vi "Measurement UI.vi"() -> ()   [LabVIEW 2022 SP3, in "Stepped Frequency Sweep_Class D Amplifier_UI.lvlib"]
uses:
  Stepped Frequency Sweep_Class D Amplifier_UI.lvlib
  shared/controls/sweep profile.ctl
  shared/controls/units - snr.ctl
  shared/controls/units - ratio.ctl
  shared/controls/digital output level units.ctl
  shared/ui/controls/view.ctl
  shared/controls/regulation target.ctl
  shared/controls/regulation target value units.ctl
  UI State.ctl
  <vilib>/Utility/miscctls.llb/LVBoundsTypeDef.ctl
  <vilib>/Utility/miscctls.llb/LVPoint32TypeDef.ctl
  <vilib>/Utility/miscctls.llb/LVPointTypeDef.ctl
  Y axis data selection.ctl
  shared/ui/UI Helpers.lvlib
  shared/audio popup ui/Audio Popup UI.lvlib
  shared/controls/audio controls.lvlib
panel:
  in  "view legend":T1
  out "plot point":string
  out "Sweep graph":cluster{"frequency (Hz)":dbl[], "THD+N":dbl[]}[](graph)
  out "Time domain graph":waveform(dbl)(graph)
  out "Frequency domain graph":T2(graph)
  in  "digital serial cfg file":string
  out "amplitude (Vrms)":dbl[](array[numeric])
  out "output power (W)":dbl[](array[numeric])
  out "SFDR (dBc)":dbl[](array[numeric])
  out "gain":dbl[](array[numeric])
  out "dynamic range (dB)":dbl[](array[numeric])
  out "THD":dbl[](array[numeric])
  out "THD+N":dbl[](array[numeric])
  out "SNR":dbl[](array[numeric])
  out "amplitude (dBFS)":dbl[](array[numeric])
  out "frequency (Hz)":dbl[](array[numeric])
  in  "Configuration tab":T3(tab)
  out "digital serial file name":string
  in  "configure digital serial":bool
  in  "master clock channel list":string caption="Master Clock Channel"
  in  "digital channel list":string caption="Digital Audio Channel"
  in  "output level":dbl=-1.0 caption="Output level" format="%#_3f"
  in  "output level units":T4
  in  "min settling cycles":u32 caption="Minimum settling cycles"
  in  "min settling time (s)":dbl=0.1 caption="Minimum settling time" format="%#_6ps"
  in  "sweep profile":T5=enum."Logarithmic" caption="Profile"
  in  "number of steps":u32=20000 caption="Number of steps"
  in  "sweep start frequency (Hz)":dbl=20.0 caption="Sweep start" format="%#_6pHz"
  in  "sweep stop frequency (Hz)":dbl=20000.0 caption="Sweep stop" format="%#_6pHz"
  in  "min measurement cycles":u32 caption="Minimum measurement cycles"
  in  "Acquisition channel":tag
  in  "acq sampling rate":dbl=51200.0 caption="Sample rate" format="%#.6pHz"
  in  "min measurement time (s)":dbl=0.1 caption="Minimum measurement time" format="%#_6ps"
  in  "lowpass filter":T6(ring) caption="Lowpass filter"
  in  "highpass filter":enum32{"DC", "AC"}(ring) caption="Highpass filter"
  in  "band start":dbl=20.0 caption="Band start" format="%#_6pHz"
  in  "band stop":dbl=20000.0 caption="Band stop" format="%#_6pHz"
  in  "weighting filter":T7(ring)=enum."A-weighting" caption="Weighting filter"
  in  "load impedance":dbl=4.0 caption="Load impedance" format="%#_6p Ohms"
  in  "output range (pk-pk)":dbl=15.0 caption="Output range" format="%.3p Vpk-pk"
  in  "regulation stop level":dbl=90.0 caption="Stop Level"
  in  "regulation output level units (stop)":T4
  in  "regulation target value units":T8 caption="Units"
  in  "regulation target value":dbl=20.0 caption="Target Value"
  in  "regulation target":T9 caption="Regulate"
  in  "enable regulation":bool caption="Enable Regulation"
  in  "regulation number of steps":u32=2 caption="Number of steps"
  in  "regulation start level":dbl=10.0 caption="Start Level"
  in  "regulation output level units":T4
  in  "gain units":T10 caption="Gain"
  in  "THD units":T10 caption="THD"
  in  "THD+N units":T10 caption="THD+N"
  in  "SNR units":T11 caption="SNR"
  in  "x-axis mapping":enum32{"linear", "logarithmic"}(ring) caption="X-axis mapping"
  in  "y-axis mapping":enum32{"linear", "logarithmic"}(ring) caption="Y-axis mapping"
  in  "channel 0 offset":u32=1
  out "fft - data":dbl[](array[numeric])
  out "fft - df":dbl
  out "fft - f0":dbl
  out "wfm - data":dbl[](array[numeric])
  out "wfm - dt":dbl
  out "wfm - t0":dbl
  out "channel name":string
  in  "acq channel":string="PXI1Slot4/ai0"
  in  "signal phase":dbl caption="phase"
  # "hidden controls - used to sync with MeasLink"
  # "hidden indicators"
  # "Digital Serial Settings"
  # "Harware Resource"
  # "Sweep"
  # "Filters"
  # "Output"
  # "Acquisition"
  # "Regulation"
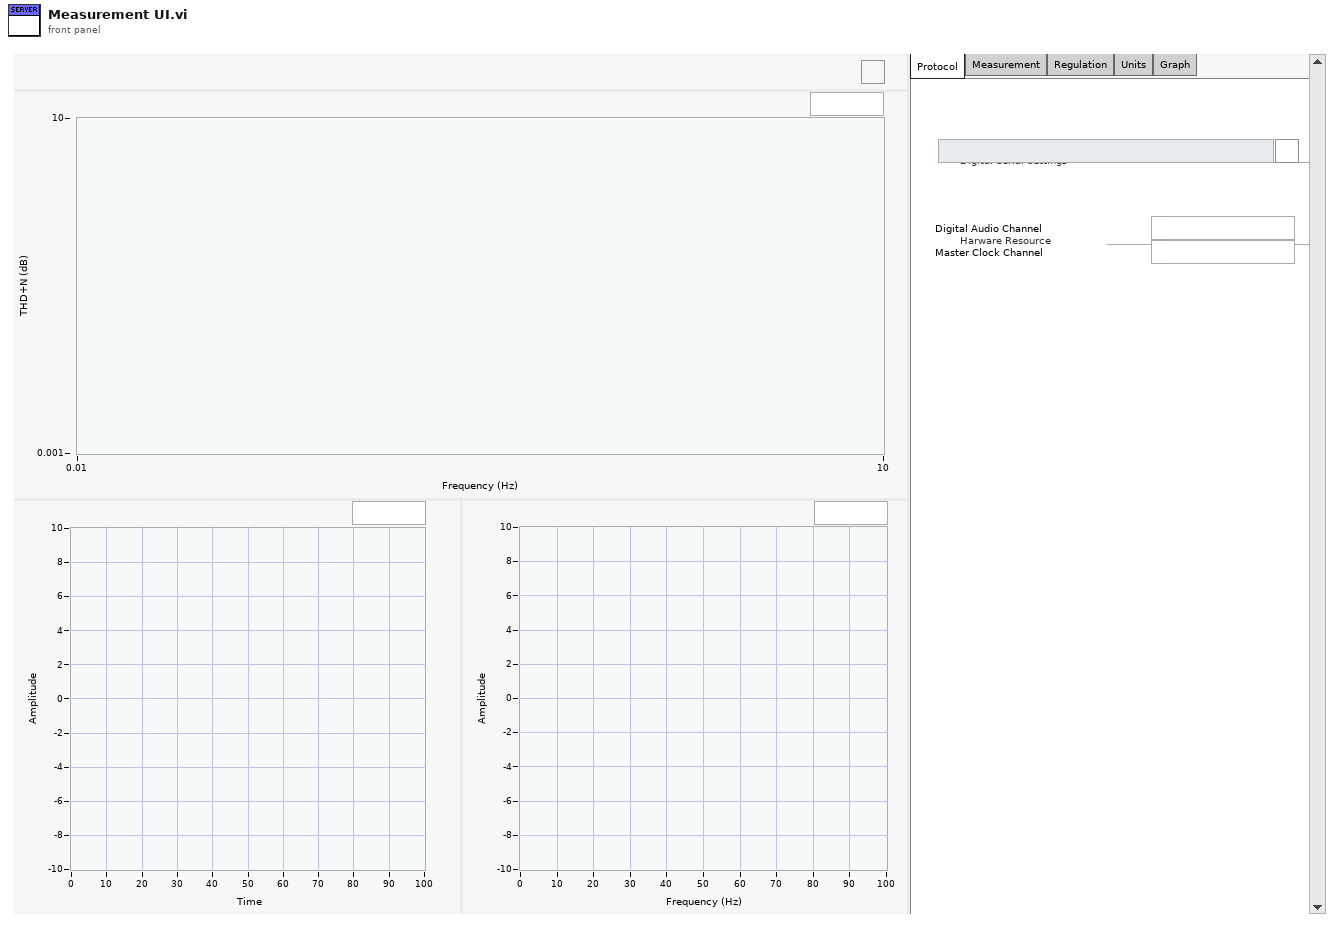
[diagram p1: front panel]
types:
  T1 = typedef "UI Helpers.lvlib/view.ctl" = bool
  T2 = cluster{"fft - f0":dbl, "fft - df":dbl, "fft - data":dbl[]}
  T3 = enum32{"Protocol", "Measurement", "Regulation", "Units", "Graph"}
  T4 = typedef "audio controls.lvlib/digital output level units.ctl" = enum32{"% FS", "dBFS", "V"}
  T5 = typedef "audio controls.lvlib/sweep profile.ctl" = enum32{"Linear", "Logarithmic"}
  T6 = enum32{"No filter", "AES17 20kHz", "AES17 40kHz"}
  T7 = enum32{"Linear", "A-weighting", "B-weighting", "C-weighting"}
  T8 = typedef "regulation target value units.ctl" = enum32{"%", "W"}
  T9 = typedef "regulation target.ctl" = enum32{"THD+N Ratio", "Output Power"}
  T10 = typedef "audio controls.lvlib/units - ratio.ctl" = enum32{"dB", "%", "x/y"}
  T11 = typedef "audio controls.lvlib/units - snr.ctl" = enum32{"dB", "x/y"}
  T12 = typedef "Stepped Frequency Sweep_Class D Amplifier_UI.lvlib/UI State.ctl" = cluster{"Graph Size":T13, "Legend Visible":bool, "Mouse Coords":T14, "Visible Plot Id":i32, "PostUI event occurred":bool, "digital serial cfg file":path}
  T13 = typedef "LVBoundsTypeDef.ctl" = cluster{"Width":u32, "Height":u32}
  T14 = typedef "LVPoint32TypeDef.ctl" = cluster{"Horizontal":i32, "Vertical":i32}
  T15 = typedef "LVPointTypeDef.ctl" = cluster{"Horizontal":i16, "Vertical":i16}
  T16 = typedef "Stepped Frequency Sweep_Class D Amplifier_UI.lvlib/Y axis data selection.ctl" = enum32{"THD+N", "THD", "SNR", "Gain", "Amplitude (dBFS)", "Amplitude (Vrms)", "Output Power (W)", "Dynamic Range (dB)", "SFDR (dBc)"}
  T17 = typedef "Audio Popup UI.lvlib/audio settings.ctl" = cluster{"digital serial file":string}
  T18 = cluster{"frequency (Hz)":dbl[], "amplitude (dBFS)":dbl[]}
  T19 = cluster{"frequency (Hz)":dbl[], "amplitude (Vrms)":dbl[]}
  T20 = cluster{"frequency (Hz)":dbl[], "output power (W)":dbl[]}
  T21 = cluster{"frequency (Hz)":dbl[], "dynamic range (dB)":dbl[]}
  T22 = cluster{"frequency (Hz)":dbl[], "SFDR (dBc)":dbl[]}
  T23 = cluster{"frequency (Hz)":dbl[], "SFDR (dBc)":dbl[]}[]
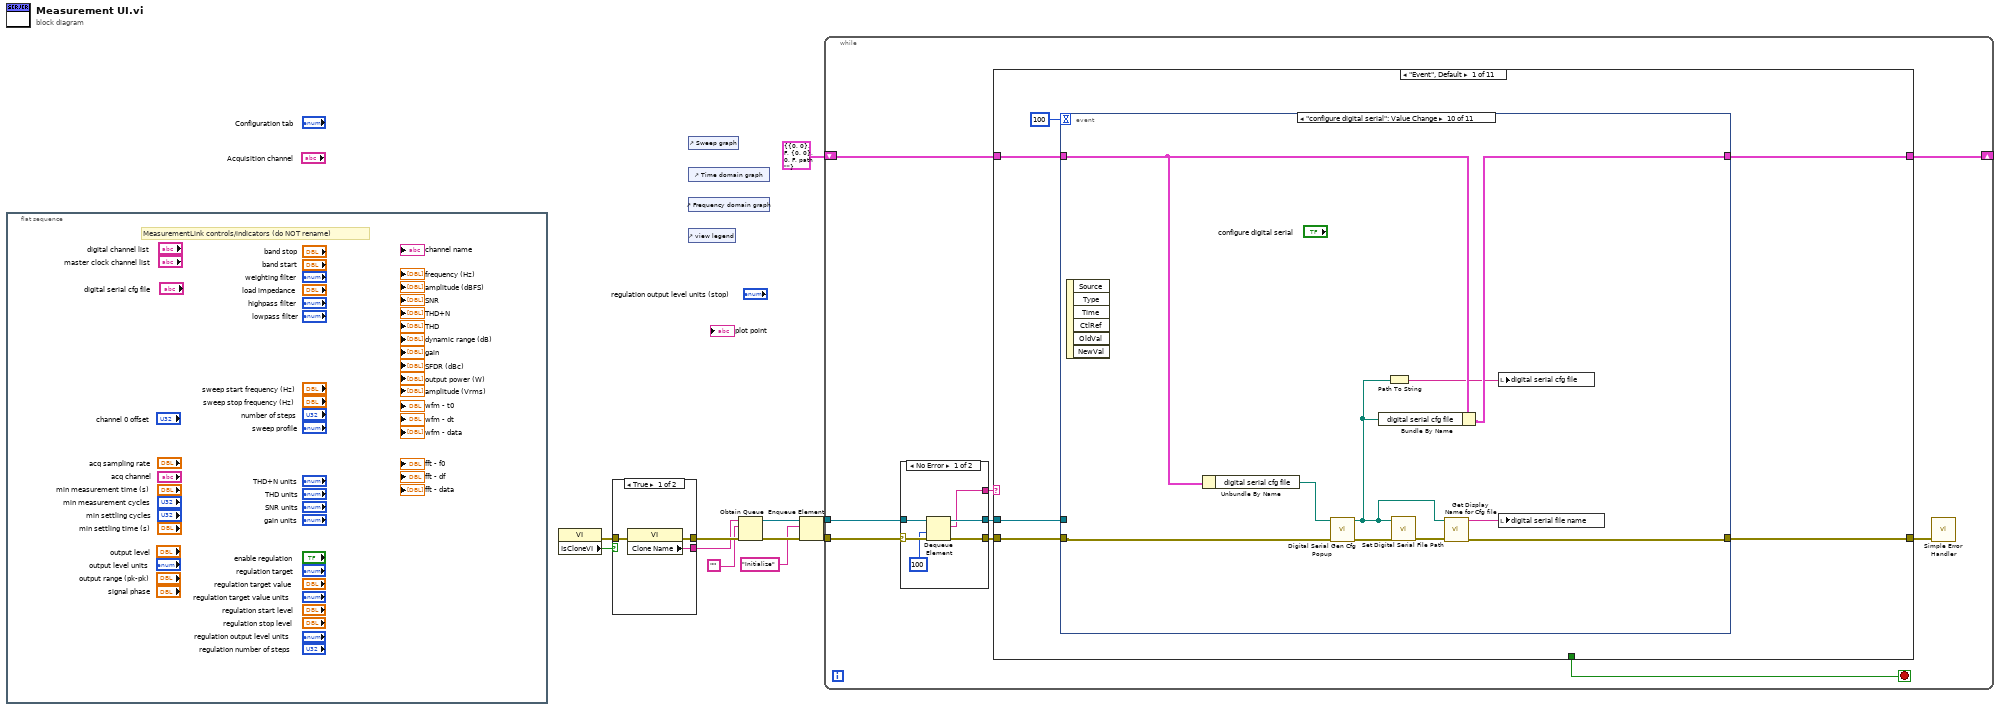
[diagram p0: block diagram]
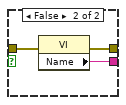
[diagram p2: hidden frame]
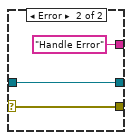
[diagram p3: hidden frame]
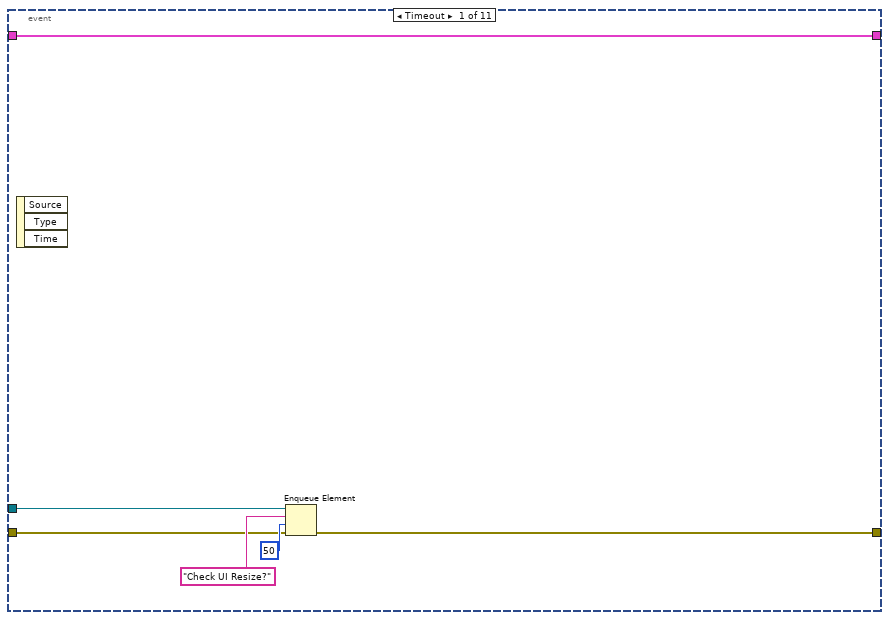
[diagram p4: hidden frame]
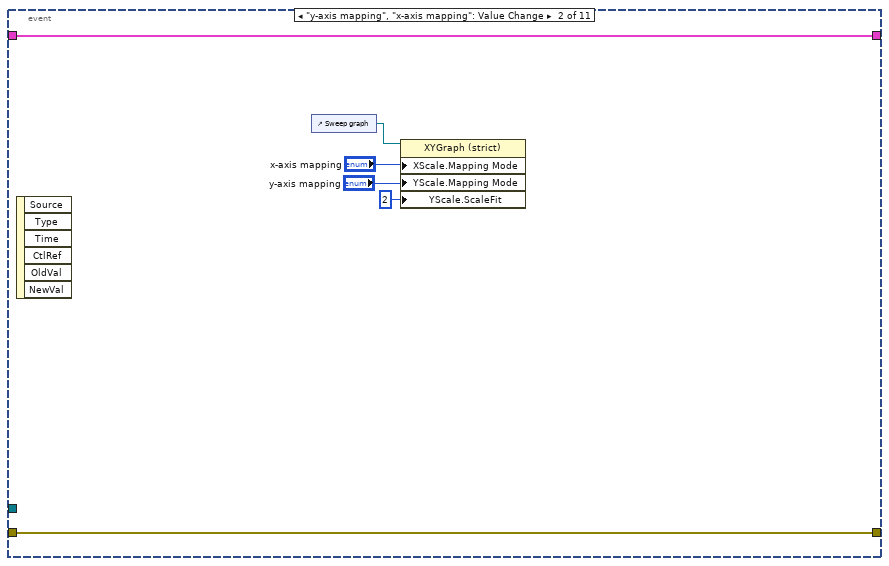
[diagram p5: hidden frame]
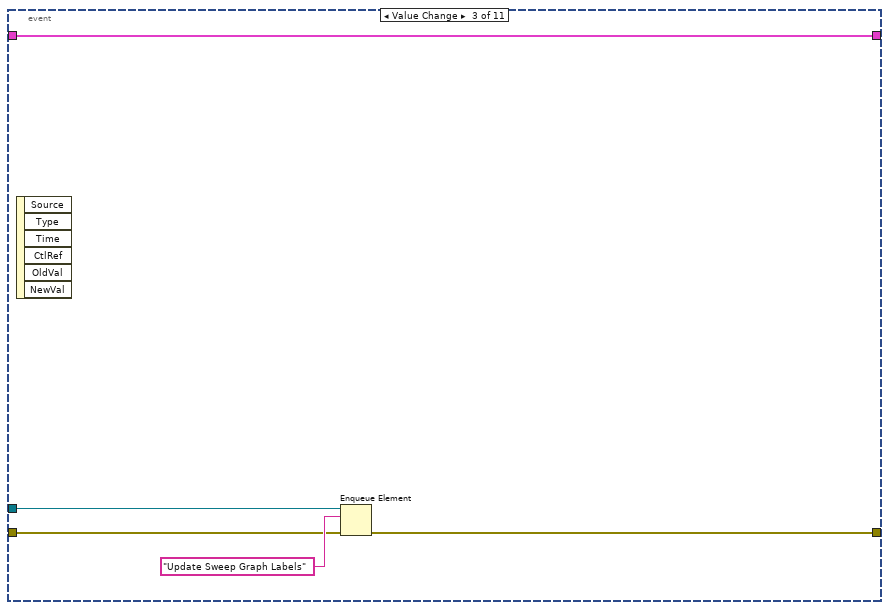
[diagram p6: hidden frame]
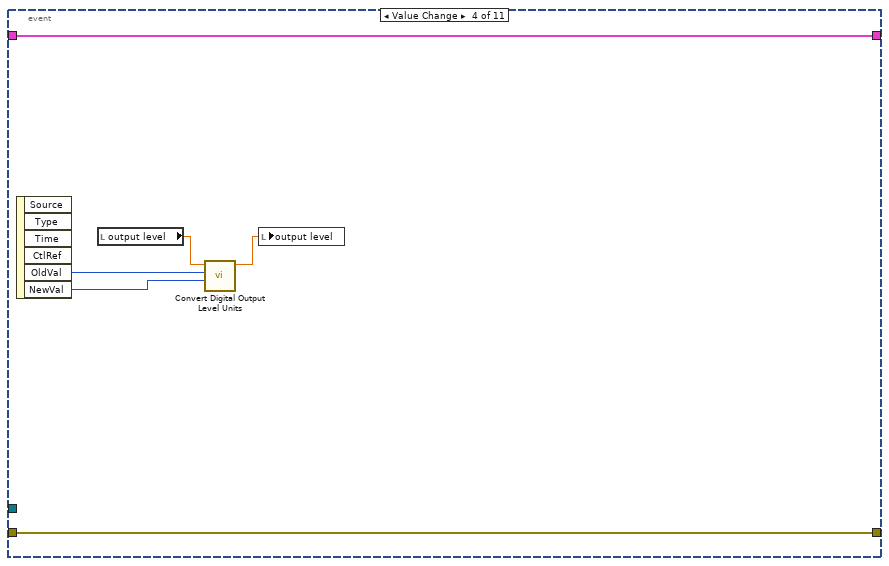
[diagram p7: hidden frame]
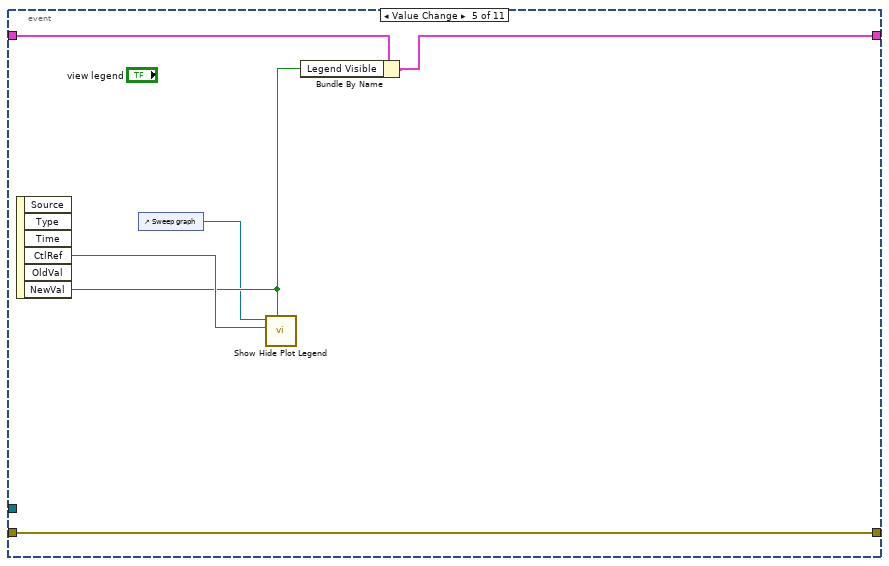
[diagram p8: hidden frame]
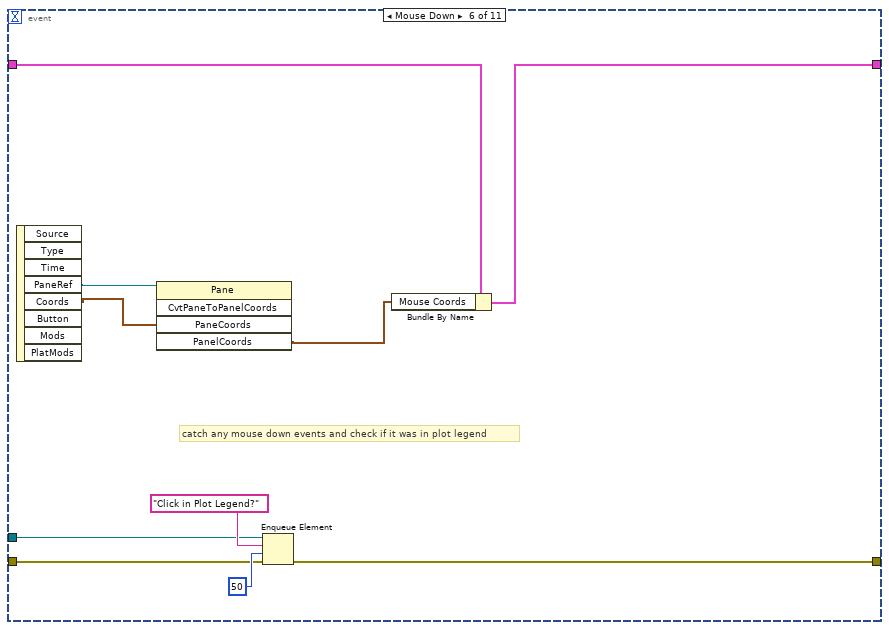
[diagram p9: hidden frame]
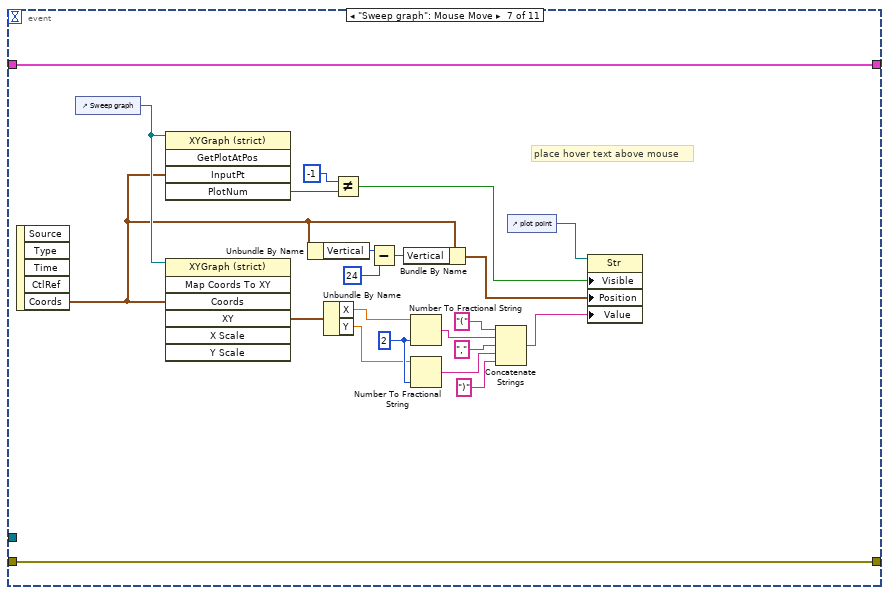
[diagram p10: hidden frame]
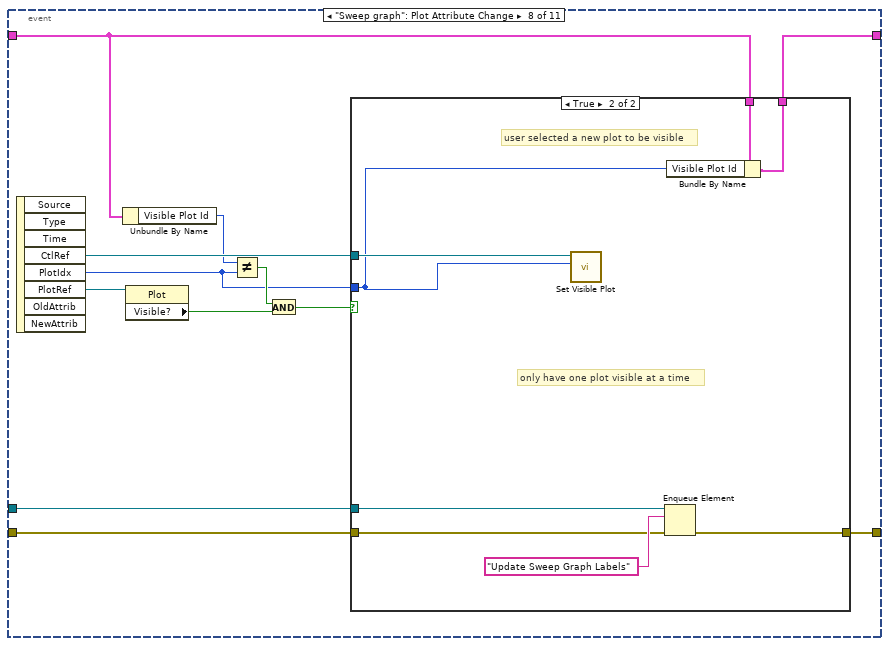
[diagram p11: hidden frame]
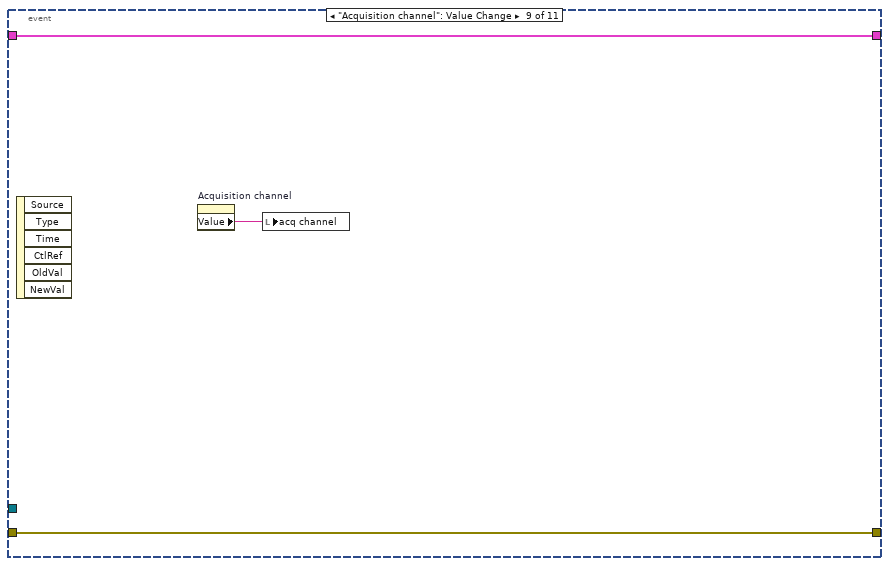
[diagram p13: hidden frame]
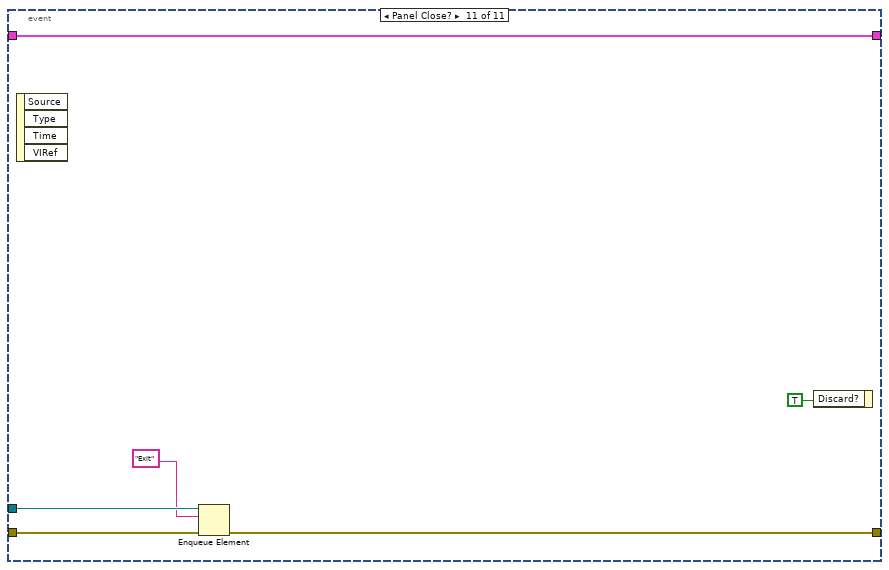
[diagram p14: hidden frame]
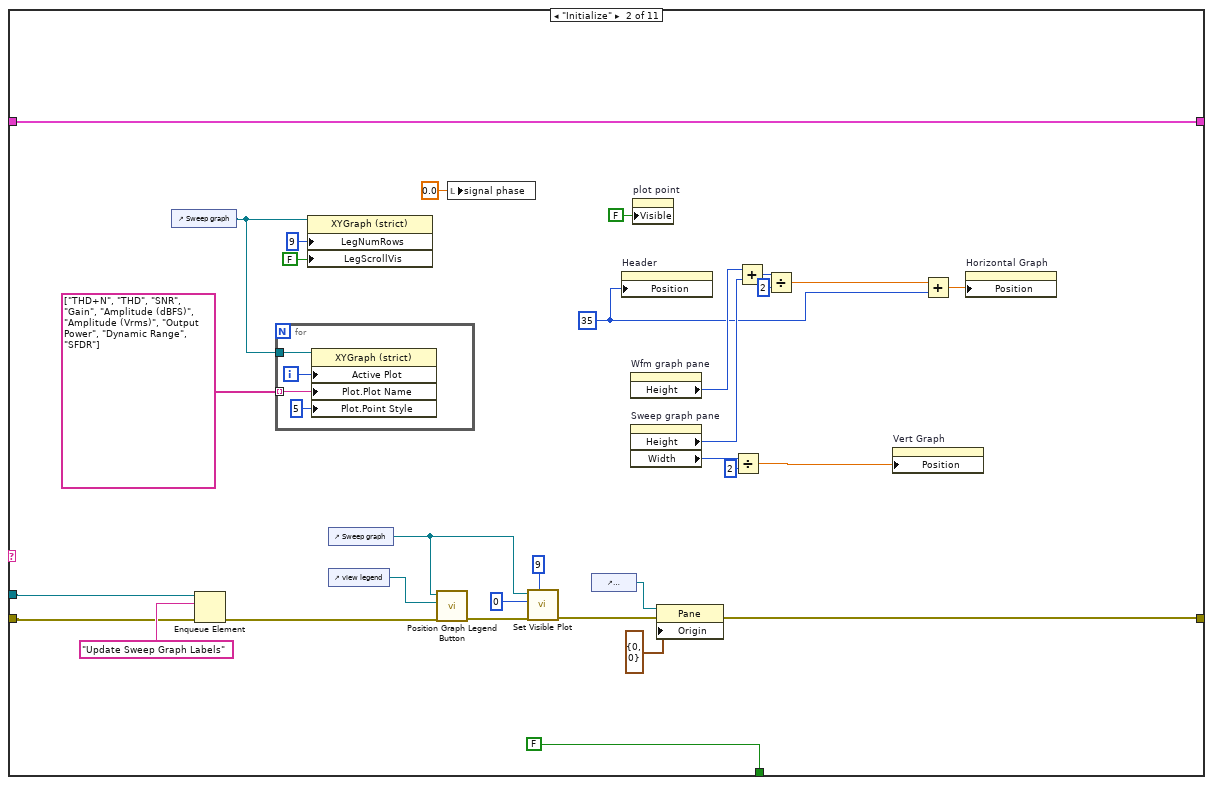
[diagram p15: hidden frame]
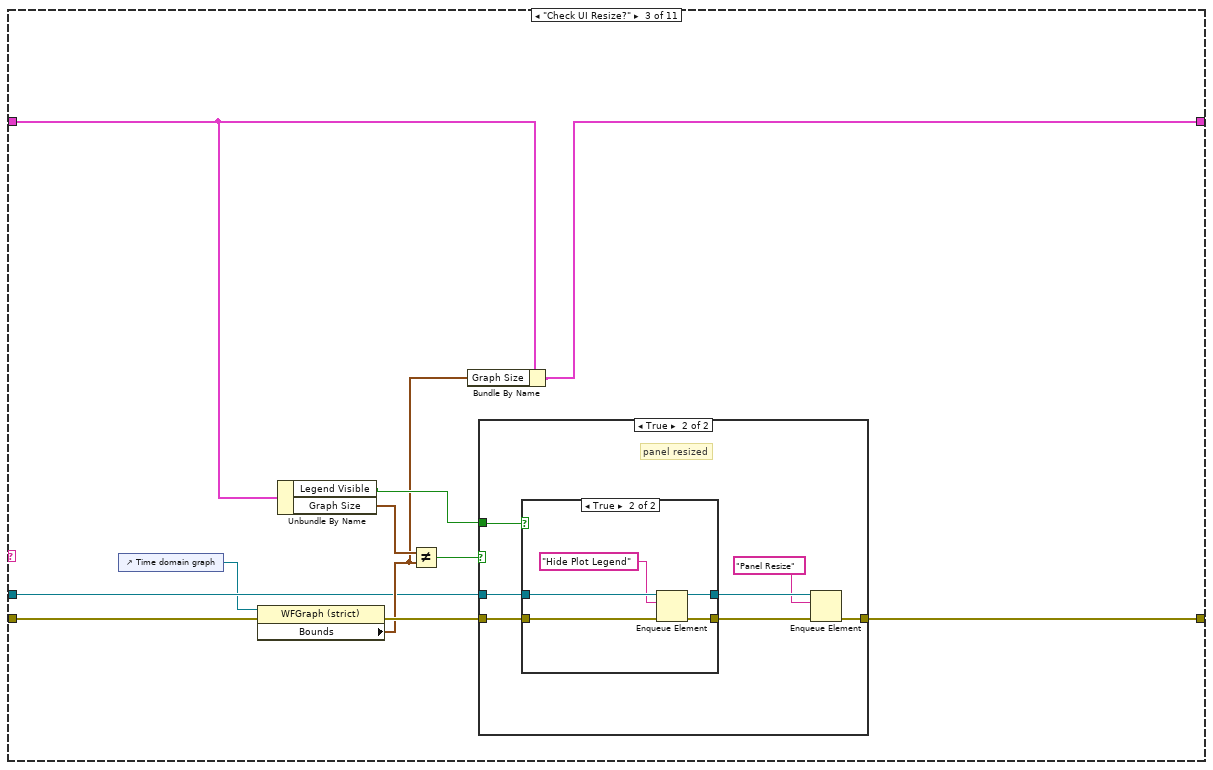
[diagram p16: hidden frame]
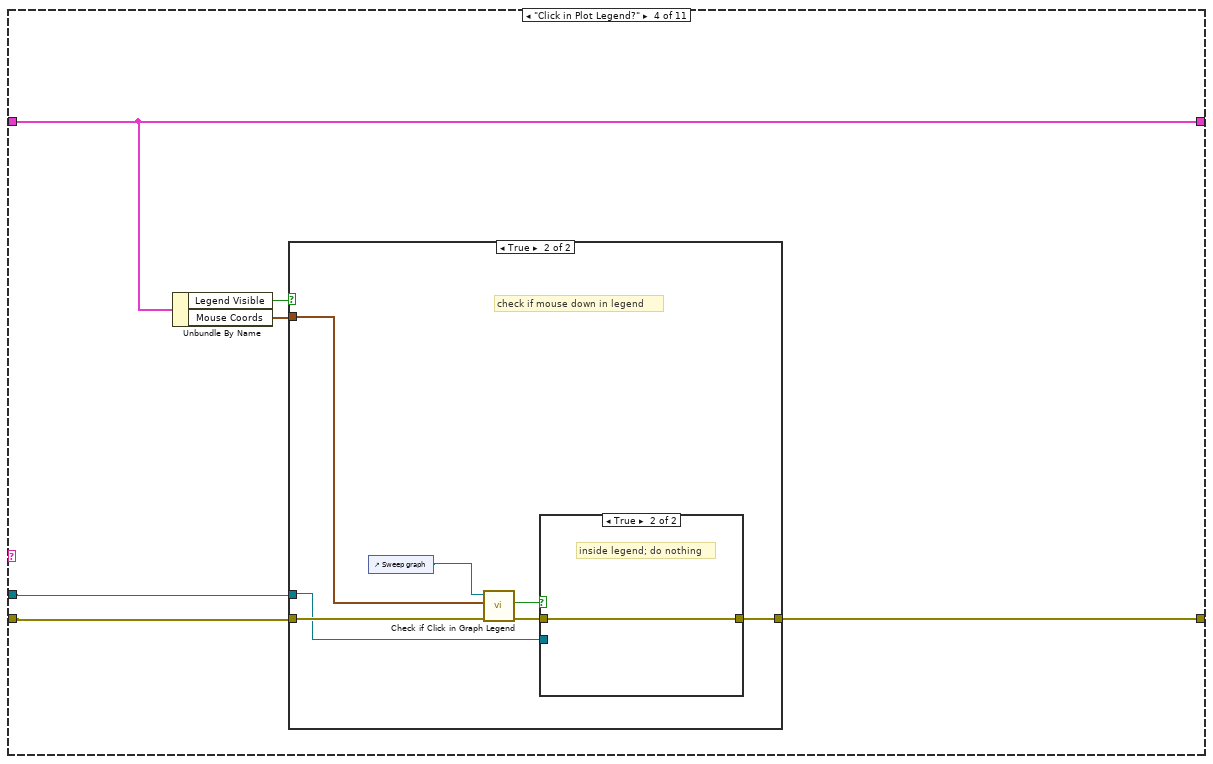
[diagram p19: hidden frame]
diagram:
  n1 = flat-sequence {
    frame #0 {
      # "MeasurementLink controls/indicators (do NOT rename)"
    }
  }
  n2 = property class="VI"() -> (error out=w2:errorcluster, "IsCloneVI"=w3:bool)  [unwired: 2 in, 1 out]
  n3 = case shown="True" w3 {
    tunnel: [w14 w17] -> w11
    tunnel: [w13 w16] -> w10
    tunnel: w2 -> [w12 w15]
    frame True {
      n4 = property class="VI"(error in=w12) -> (error out=w14:errorcluster, "Clone Name"=w13:string)  [unwired: 1 in, 1 out]
    }
    frame False {
      n5 = property class="VI"(error in=w15) -> (error out=w17:errorcluster, "Name"=w16:string)  [unwired: 1 in, 1 out]
    }
  }
  n6 = control-ref of="Sweep graph"() -> ()  [unwired: 1 out]
  n7 = control-ref of="Time domain graph"() -> ()  [unwired: 1 out]
  n8 = control-ref of="Frequency domain graph"() -> ()  [unwired: 1 out]
  n9 = control-ref of="view legend"() -> ()  [unwired: 1 out]
  n10 = Obtain Queue(name (unnamed)=w10, element data type="", error in (no error)=w11) -> (queue out=w7:refnum<queue>, error out=w9:errorcluster)  [unwired: 2 in, 1 out]
  n11 = Enqueue Element(queue=w7, element="Initialize", error in (no error)=w9) -> (queue out=w6:refnum<queue>, error out=w8:errorcluster)  [unwired: 1 in, 1 out]
  n12 = while {
    tunnel: w6 -> [w24]
    shift-right: [w20] -> _
    shift-left: T12 {"Graph Size"={"Width"=0, "Height"=0}, "Legend Visible"=FALSE, "Mouse Coords"={"Horizontal"=0, "Vertical"=0}, "Visible Plot Id"=0, "PostUI event occurred"=FALSE, "digital serial cfg file"=path ""} ("UI State") -> [w19]
    tunnel: w8 -> [w26]
    stop <- w21 stop-if-true
    n13 = case shown="No Error" w26 {
      selector: w26 -> [w32 w35]
      tunnel: [w31 w35] -> w25
      tunnel: w24 -> [w30 w34]
      tunnel: [w29 w34] -> w23
      tunnel: [w28 "Handle Error"] -> w22
      frame No Error {
        n14 = Dequeue Element(queue=w30, timeout in ms (-1)=100, error in (no error)=w32) -> (queue out=w29:refnum<queue>, element=w28:string, error out=w31:errorcluster)  [unwired: 1 out]
      }
      frame Error {
      }
    }
    n15 = case shown="\"Event\", Default" w22 {
      tunnel: w25 -> [w40 w152 w183 w207 w227 w235 w243 w291 w303 w316 w318]
      tunnel: w23 -> [w38 w153 w184 w208 _ _ w242 _ _ w314 _]
      tunnel: [w41 w148 w182 w206 w226 w234 w237 w291 w303 w311 w318] -> w18
      tunnel: [_ FALSE _ _ _ _ _ _ _ TRUE _] -> w21
      tunnel: [w36 w144 w179 w205 w229 w236 w240 w290 w302 w309 w317] -> w20
      tunnel: w19 -> [w37 w144 w180 w205 w230 w236 w241 w290 w302 w309 w317]
      frame "Event", Default {
        n16 = event shown="[9] \"configure digital serial\": Value Change" {
          selector: _ -> [_ _ _ _ _ _ _ _ _ _ _]
          dyn-events: _ -> [_ _ _ _ _ _ _ _ _ _ _]
          timeout: 100 -> [_ _ _ _ _ _ _ _ _ _ _]
          tunnel: [w44 w48 w54 w59 w70 w76 w102 w110 w125 w132 w141] -> w41
          tunnel: w40 -> [w45 w48 w55 w59 w70 w78 w102 w112 w125 w133 w142]
          tunnel: w38 -> [w43 _ w56 _ _ w77 _ w111 _ _ w140]
          tunnel: w37 -> [w42 w49 w58 w60 w67 w75 w101 w105 w126 w131 w138]
          tunnel: [w42 w49 w58 w60 w66 w74 w101 w104 w126 w130 w138] -> w36
          event Timeout {
            n17 = event-data() -> ()  [unwired: 1 in, 3 out]
            n18 = Enqueue Element(queue=w43, element="Check UI Resize?", timeout in ms (-1)=50, error in (no error)=w45) -> (error out=w44:errorcluster)  [unwired: 2 out]
          }
          event "y-axis mapping", "x-axis mapping": Value Change {
            n19 = event-data() -> ()  [unwired: 1 in, 6 out]
            n20 = control-ref of="Sweep graph"() -> (w51:refnum<vi>)
            n21 = property on="Property Node" class="XYGraph (strict)"(reference=w51, "XScale.Mapping Mode"="x-axis mapping", "YScale.Mapping Mode"="y-axis mapping", "YScale.ScaleFit"=u8 2 ("Y Scale.Scale Fit")) -> ()  [unwired: 1 in, 2 out]
          }
          event Value Change {
            n22 = event-data() -> ()  [unwired: 1 in, 6 out]
            n23 = Enqueue Element(queue=w56, element="Update Sweep Graph Labels", error in (no error)=w55) -> (error out=w54:errorcluster)  [unwired: 1 in, 2 out]
          }
          event Value Change {
            n24 = event-data() -> ("OldVal"=w64:T4, "NewVal"=w63:T4)  [unwired: 1 in, 4 out]
            n25 = local read "output level"() -> (w61:dbl)
            n26 = call "Convert Digital Output Level Units.vi"("new output level units"=w63, "previous output level units"=w64, "previous output level"=w61) -> ("new output level"=w62:dbl)  [unwired: 8 in]
            n27 = local write "output level"(w62) -> ()
          }
          event Value Change {
            n28 = event-data() -> ("CtlRef"=w69:refnum<vi>, "NewVal"=w68:T1)  [unwired: 1 in, 4 out]
            n29 = control-ref of="Sweep graph"() -> (w65:refnum<vi>)
            n30 = call "Show Hide Plot Legend.vi"("show"=w68, "view reference"=w69, "graph reference"=w65) -> ()  [unwired: 8 in, 1 out]
            n31 = Bundle By Name(cluster=w67, "Legend Visible"=w68) -> (w66:T12)
          }
          event Mouse Down {
            # "catch any mouse down events and check if it was in plot legend"
            n32 = event-data() -> ("PaneRef"=w73:refnum<vi>, "Coords"=w72:T14)  [unwired: 1 in, 6 out]
            n33 = invoke class="Pane" method="CvtPaneToPanelCoords"(reference=w73, "PaneCoords"=w72) -> ("PanelCoords"=w71:T15)  [unwired: 3 in, 4 out]
            n34 = Enqueue Element(queue=w77, element="Click in Plot Legend?", timeout in ms (-1)=50, error in (no error)=w78) -> (error out=w76:errorcluster)  [unwired: 2 out]
            n35 = Bundle By Name(cluster=w75, "Mouse Coords"=w71) -> (w74:T12)
          }
          event "Sweep graph": Mouse Move {
            w91 = i16 2 ("precision (6)")
            # "place hover text above mouse"
            n36 = event-data() -> ("Coords"=w86:T14)  [unwired: 1 in, 4 out]
            n37 = control-ref of="Sweep graph"() -> (w87:refnum<vi>)
            n38 = invoke class="XYGraph (strict)" method="GetPlotAtPos"(reference=w87, "InputPt"=w86) -> ("PlotNum"=w99:i32)  [unwired: 3 in, 4 out]
            n39 = invoke class="XYGraph (strict)" method="Map Coords To XY"(reference=w87, "Coords"=w86) -> ("XY"=w100:cluster{"X":dbl, "Y":dbl})  [unwired: 5 in, 6 out]
            n40 = Unbundle By Name(w86) -> ("Vertical"=w84:i32)
            n41 = Unbundle By Name(w100) -> ("X"=w89:dbl, "Y"=w88:dbl)
            n42 = Not Equal?(x=-1, y=w99) -> (x != y?=w97:bool)
            n43 = Subtract(x=w84, y=24) -> (x-y=w83:i32)
            n44 = Bundle By Name(cluster=w86, "Vertical"=w83) -> (w85:T14)
            n45 = Number To Fractional String(number=w89, precision (6)=w91) -> (F-format string=w95:string)  [unwired: 2 in]
            n46 = Number To Fractional String(number=w88, precision (6)=w91) -> (F-format string=w93:string)  [unwired: 2 in]
            n47 = Concatenate Strings("(" ("string"), w95, "," ("string"), w93, ")" ("string")) -> (w90:string)
            n48 = control-ref of="plot point"() -> (w81:refnum<vi>)
            n49 = property on="Property Node" class="Str"(reference=w81, "Visible"=w97, "Position"=w85, "Value"=w90) -> ()  [unwired: 1 in, 2 out]
          }
          event "Sweep graph": Plot Attribute Change {
            n50 = event-data() -> ("CtlRef"=w113:refnum<vi>, "PlotIdx"=w103:i32, "PlotRef"=w114:refnum<vi>)  [unwired: 1 in, 5 out]
            n51 = Unbundle By Name(w105) -> ("Visible Plot Id"=w109:i32)
            n52 = property class="Plot"(reference=w114) -> ("Visible?"=w107:bool)  [unwired: 1 in, 2 out]
            n53 = Not Equal?(x=w109, y=w103) -> (x != y?=w108:bool)
            n54 = And(x=w108, y=w107) -> (x .and. y?=w106:bool)
            n55 = case shown="True" w106 {
              tunnel: w113 -> [_ w124]
              tunnel: w112 -> [w116 w122]
              tunnel: w111 -> [_ w121]
              tunnel: [w116 w120] -> w110
              tunnel: w105 -> [w115 w119]
              tunnel: [w115 w118] -> w104
              tunnel: w103 -> [_ w117]
              frame False {
              }
              frame True {
                # "only have one plot visible at a time"
                # "user selected a new plot to be visible"
                n56 = call "Set Visible Plot.vi"("Plot Id"=w117, "XYGraph in"=w124) -> ()  [unwired: 9 in, 1 out]
                n57 = Enqueue Element(queue=w121, element="Update Sweep Graph Labels", error in (no error)=w122) -> (error out=w120:errorcluster)  [unwired: 1 in, 2 out]
                n58 = Bundle By Name(cluster=w119, "Visible Plot Id"=w117) -> (w118:T12)
              }
            }
          }
          event "Acquisition channel": Value Change {
            n59 = event-data() -> ()  [unwired: 1 in, 6 out]
            n60 = property on="Acquisition channel" class="DAQmxName"() -> ("Value"=w127:string)  [unwired: 2 in, 2 out]
            n61 = local write "acq channel"(w127) -> ()
          }
          event "configure digital serial": Value Change {
            n62 = event-data() -> ()  [unwired: 1 in, 6 out]
            n63 = Unbundle By Name(w131) -> ("digital serial cfg file"=w137:path)
            n64 = call "Digital Serial Gen Cfg Popup.vi"("error in (no error)"=w133, "config file in"=w137) -> ("error out"=w136:errorcluster, "config file out"=w134:path)  [unwired: 7 in, 1 out]
            n65 = Bundle By Name(cluster=w131, "digital serial cfg file"=w134) -> (w130:T12)
            n66 = Path To String(path=w134) -> (string=w128:string)
            n67 = call "Set Digital Serial File Path.vi"("error in (no error)"=w136, "digital serial file"=w134) -> ("error out"=w135:errorcluster)  [unwired: 9 in]
            n68 = call "Get Display Name for Cfg file.vi"("error in (no error)"=w135, "file path"=w134) -> ("error out"=w132:errorcluster, "display string"=w129:string)  [unwired: 8 in]
            n69 = local write "digital serial cfg file"(w128) -> ()
            n70 = local write "digital serial file name"(w129) -> ()
          }
          event Panel Close? {
            n71 = event-data() -> ()  [unwired: 1 in, 4 out]
            n72 = Enqueue Element(queue=w140, element="Exit", error in (no error)=w142) -> (error out=w141:errorcluster)  [unwired: 1 in, 2 out]
            n73 = event-data("Discard?"=TRUE) -> ()  [unwired: 1 in, 1 out]
          }
        }
      }
      frame "Initialize" {
        w150 = 35 ("Splitter Position")
        n74 = control-ref of="Sweep graph"() -> (w158:refnum<vi>)
        n75 = Enqueue Element(queue=w153, element="Update Sweep Graph Labels", error in (no error)=w152) -> (error out=w151:errorcluster)  [unwired: 1 in, 2 out]
        n76 = for {
          tunnel: string[] ["THD+N", "THD", "SNR", "Gain", "Amplitude (dBFS)", "Amplitude (Vrms)", "Output Power", "Dynamic Range", "SFDR"] -> [w177] mode=indexing
          tunnel: w158 -> [w176]
          i -> [w178]
          n77 = property on="Property Node" class="XYGraph (strict)"(reference=w176, "Active Plot"=w178, "Plot.Plot Name"=w177, "Plot.Point Style"=u8 5) -> ()  [unwired: 1 in, 2 out]
        }
        n78 = property class="XYGraph (strict)"(reference=w158, "LegNumRows"=u32 9 ("Legend:Number of Rows"), "LegScrollVis"=FALSE ("Legend:Scrollbar Visible")) -> ()  [unwired: 1 in, 2 out]
        n79 = control-ref of="Sweep graph"() -> (w161:refnum<vi>)
        n80 = control-ref of="view legend"() -> (w172:refnum<vi>)
        n81 = call "Position Graph Legend Button.vi"("error in (no error)"=w151, "view legend"=w172, "graph"=w161) -> ("error out"=w162:errorcluster)  [unwired: 8 in]
        n82 = local write "signal phase"(0.0 ("signal phase")) -> ()
        n83 = call "Set Visible Plot.vi"("number of plots"=9, "error in (no error)"=w162, "Plot Id"=0, "XYGraph in"=w161) -> ("error out"=w149:errorcluster)  [unwired: 7 in]
        n84 = control-ref of="Configuration Pane"() -> (w147:refnum<vi>)
        n85 = property on="Header" class="Splitter"("Position"=w150) -> ()  [unwired: 2 in, 2 out]
        n86 = property on="Wfm graph pane" class="Pane"() -> ("Height"=w165:u32)  [unwired: 2 in, 2 out]
        n87 = property on="Sweep graph pane" class="Pane"() -> ("Height"=w164:u32, "Width"=w167:u32)  [unwired: 2 in, 2 out]
        n88 = property on="plot point" class="Str"("Visible"=FALSE) -> ()  [unwired: 2 in, 2 out]
        n89 = property class="Pane"(reference=w147, error in=w149, "Origin"=T15 {"Horizontal"=0, "Vertical"=0}) -> (error out=w148:errorcluster)  [unwired: 1 out]
        n90 = Divide(x=w167, y=2) -> (x/y=w166:dbl)
        n91 = Add(x=w165, y=w164) -> (x+y=w163:u32)
        n92 = Divide(x=w163, y=2) -> (x/y=w170:dbl)
        n93 = property on="Vert Graph" class="Splitter"("Position"=w166) -> ()  [unwired: 2 in, 2 out]
        n94 = Add(x=w170, y=w150) -> (x+y=w169:dbl)
        n95 = property on="Horizontal Graph" class="Splitter"("Position"=w169) -> ()  [unwired: 2 in, 2 out]
      }
      frame "Check UI Resize?" {
        n96 = control-ref of="Time domain graph"() -> (w181:refnum<vi>)
        n97 = property on="Property Node" class="WFGraph (strict)"(reference=w181, error in=w183) -> (error out=w189:errorcluster, "Bounds"=w185:T13)  [unwired: 1 out]
        n98 = Unbundle By Name(w180) -> ("Legend Visible"=w187:bool, "Graph Size"=w186:T13)
        n99 = Not Equal?(x=w186, y=w185) -> (x != y?=w188:bool)
        n100 = Bundle By Name(cluster=w180, "Graph Size"=w185) -> (w179:T12)
        n101 = case shown="True" w188 {
          tunnel: w189 -> [w190 w197]
          tunnel: [w190 w192] -> w182
          tunnel: w187 -> [_ w195]
          tunnel: w184 -> [_ w196]
          frame False {
            # "no resize"
          }
          frame True {
            # "panel resized"
            n102 = case shown="True" w195 {
              tunnel: w197 -> [w199 w204]
              tunnel: [w199 w203] -> w194
              tunnel: w196 -> [w198 w202]
              tunnel: [w198 w200] -> w193
              frame False {
              }
              frame True {
                n103 = Enqueue Element(queue=w202, element="Hide Plot Legend", error in (no error)=w204) -> (queue out=w200:refnum<queue>, error out=w203:errorcluster)  [unwired: 1 in, 1 out]
              }
            }
            n104 = Enqueue Element(queue=w193, element="Panel Resize", error in (no error)=w194) -> (error out=w192:errorcluster)  [unwired: 1 in, 2 out]
          }
        }
      }
      frame "Click in Plot Legend?" {
        n105 = Unbundle By Name(w205) -> ("Legend Visible"=w209:bool, "Mouse Coords"=w210:T14)
        n106 = case shown="True" w209 {
          tunnel: w210 -> [_ w217]
          tunnel: w208 -> [_ w214]
          tunnel: w207 -> [w211 w218]
          tunnel: [w211 w213] -> w206
          frame False {
            # "legend not visible; do nothing"
          }
          frame True {
            # "check if mouse down in legend"
            n107 = control-ref of="Sweep graph"() -> (w212:refnum<vi>)
            n108 = call "Check if Click in Graph Legend.vi"("error in (no error)"=w218, "Mouse Coords"=w217, "WaveformGraph"=w212) -> ("error out"=w215:errorcluster, "click in legend?"=w216:bool)  [unwired: 7 in]
            n109 = case shown="True" w216 {
              tunnel: w215 -> [w222 w223]
              tunnel: w214 -> [w221 _]
              tunnel: [w220 w223] -> w213
              frame False {
                n110 = Enqueue Element(queue=w221, element="Hide Plot Legend", error in (no error)=w222) -> (error out=w220:errorcluster)  [unwired: 1 in, 2 out]
              }
              frame True {
                # "inside legend; do nothing"
              }
            }
          }
        }
      }
      frame "Hide Plot Legend" {
        n111 = control-ref of="Sweep graph"() -> (w224:refnum<vi>)
        n112 = control-ref of="view legend"() -> (w225:refnum<vi>)
        n113 = call "Show Hide Plot Legend.vi"("show"=FALSE, "error in (no error)"=w227, "view reference"=w225, "graph reference"=w224) -> ("error out"=w226:errorcluster)  [unwired: 7 in]
        n114 = Bundle By Name(cluster=w230, "Legend Visible"=FALSE ("legend visible")) -> (w229:T12)
      }
      frame "Panel Resize" {
        n115 = control-ref of="Sweep graph"() -> (w233:refnum<vi>)
        n116 = control-ref of="view legend"() -> (w232:refnum<vi>)
        n117 = call "Position Graph Legend Button.vi"("error in (no error)"=w235, "view legend"=w232, "graph"=w233) -> ("error out"=w234:errorcluster)  [unwired: 8 in]
      }
      frame "Post UI Update" {
        # "This case will be triggered, after framework updates the User interface with result values."
        n118 = for {
          tunnel: w242 -> [w267]
          shift-right: [w266] -> w238
          shift-left: w243 -> [w268]
          tunnel: string[] ["Update Graphs"] -> [w265] mode=indexing
          n119 = Enqueue Element(queue=w267, element=w265, timeout in ms (-1)=50, error in (no error)=w268) -> (error out=w266:errorcluster)  [unwired: 2 out]
        }
        n120 = Unbundle By Name(w241) -> ("PostUI event occurred"=w239:bool)
        n121 = case shown="False" w239 {
          tunnel: w241 -> [w254 w264]
          tunnel: [w253 w264] -> w240
          tunnel: w238 -> [w251 w263]
          tunnel: [w249 w263] -> w237
          frame False {
            # "do this on first PostUI Event (happens when panel loads)"
            # "Initialize the DAQmx channel control"
            n122 = local read "digital serial cfg file"() -> (w246:string)
            n123 = local read "acq channel"() -> (w256:string)
            n124 = Empty String/Path?(string/path=w246) -> (empty?=w252:bool)
            n125 = case shown="True" w252 {
              tunnel: w251 -> [w258 w262]
              tunnel: [w258 w260] -> w250
              tunnel: w246 -> [w257 _]
              tunnel: [w257 w259] -> w248
              frame False {
              }
              frame True {
                n126 = call "Get Audio Settings.vi"("error in (no error)"=w262) -> ("error out"=w260:errorcluster, "audio settings"=w261:T17)  [unwired: 9 in]
                n127 = Unbundle By Name(w261) -> ("digital serial file"=w259:string)
              }
            }
            n128 = property on="Acquisition channel" class="DAQmxName"("Value"=w256) -> ()  [unwired: 2 in, 2 out]
            n129 = String To Path(string=w248) -> (path=w247:path)
            n130 = call "Get Display Name for Cfg file.vi"("error in (no error)"=w250, "file path"=w247) -> ("error out"=w249:errorcluster, "display string"=→"digital serial file name":string)  [unwired: 8 in]
            n131 = local write "digital serial cfg file"(w248) -> ()
            n132 = Bundle By Name(cluster=w254, "PostUI event occurred"=TRUE, "digital serial cfg file"=w247) -> (w253:T12)
          }
          frame True {
          }
        }
      }
      frame "Update Graphs" {
        n133 = local read "wfm - data"() -> (w297:dbl[])
        n134 = local read "fft - data"() -> (w294:dbl[])
        n135 = local read "wfm - dt"() -> (w296:dbl)
        n136 = local read "fft - df"() -> (w293:dbl)
        n137 = local read "fft - f0"() -> (w292:dbl)
        n138 = local read "dynamic range (dB)"() -> (w279:dbl[])
        n139 = local read "output power (W)"() -> (w280:dbl[])
        n140 = local read "amplitude (Vrms)"() -> (w281:dbl[])
        n141 = local read "amplitude (dBFS)"() -> (w282:dbl[])
        n142 = Bundle By Name("dt"=w296, "Y"=w297) -> (→"Time domain graph":waveform(dbl))  [unwired: 1 in]
        n143 = Bundle("fft - f0"=w292, "fft - df"=w293, "fft - data"=w294) -> (→"Frequency domain graph":T2)  [unwired: 1 in]
        n144 = local read "frequency (Hz)"() -> (w286:dbl[])
        n145 = local read "SFDR (dBc)"() -> (w278:dbl[])
        n146 = local read "THD+N"() -> (w289:dbl[])
        n147 = local read "THD"() -> (w285:dbl[])
        n148 = local read "gain"() -> (w283:dbl[])
        n149 = local read "SNR"() -> (w284:dbl[])
        n150 = Bundle("frequency (Hz)"=w286, "THD+N"=w289) -> (w288:cluster{"frequency (Hz)":dbl[], "THD+N":dbl[]})  [unwired: 1 in]
        n151 = Bundle("frequency (Hz)"=w286, "THD"=w285) -> (w277:cluster{"frequency (Hz)":dbl[], "THD":dbl[]})  [unwired: 1 in]
        n152 = Bundle("frequency (Hz)"=w286, "SNR"=w284) -> (w276:cluster{"frequency (Hz)":dbl[], "SNR":dbl[]})  [unwired: 1 in]
        n153 = Bundle("frequency (Hz)"=w286, "gain"=w283) -> (w275:cluster{"frequency (Hz)":dbl[], "gain":dbl[]})  [unwired: 1 in]
        n154 = Bundle("frequency (Hz)"=w286, "amplitude (dBFS)"=w282) -> (w274:T18)  [unwired: 1 in]
        n155 = Bundle("frequency (Hz)"=w286, "amplitude (Vrms)"=w281) -> (w273:T19)  [unwired: 1 in]
        n156 = Bundle("frequency (Hz)"=w286, "output power (W)"=w280) -> (w272:T20)  [unwired: 1 in]
        n157 = Bundle("frequency (Hz)"=w286, "dynamic range (dB)"=w279) -> (w271:T21)  [unwired: 1 in]
        n158 = Bundle("frequency (Hz)"=w286, "SFDR (dBc)"=w278) -> (w270:T22)  [unwired: 1 in]
        n159 = Build Array(w288, w277, w276, w275, w274, w273, w272, w271, w270) -> (→"Sweep graph":T23)
      }
      frame "Update Sweep Graph Labels" {
        n160 = Unbundle By Name(w302) -> ("Visible Plot Id"=w300:i32)
        n161 = local read "THD+N units"() -> (w307:T10)
        n162 = local read "THD units"() -> (w306:T10)
        n163 = local read "gain units"() -> (w305:T10)
        n164 = local read "SNR units"() -> (w308:T11)
        n165 = Type Cast(type=Y_axis_data_selection."THD+N" ("y-axis data"), x=w300) -> (*(type *) &x=w299:T16)
        n166 = call "Get Y Axis Name.vi"("gain units"=w305, "THD units"=w306, "THD+N units"=w307, "SNR units"=w308, "y-axis data"=w299) -> ("units"=w304:string)  [unwired: 6 in]
        n167 = property on="Sweep graph" class="XYGraph (strict)"("YScale.NameLbl.Text"=w304) -> ()  [unwired: 2 in, 2 out]
      }
      frame "Exit" {
        # "This case is triggered to close the User Interface from framework"
        n168 = Flush Queue(queue=w314, error in (no error)=w316) -> (queue out=w313:refnum<queue>, error out=w312:errorcluster)  [unwired: 1 out]
        n169 = Release Queue(queue=w313, force destroy? (F)=TRUE, error in (no error)=w312) -> (error out=w311:errorcluster)  [unwired: 2 out]
      }
      frame "Handle Error" {
      }
    }
    n170 = call <vilib>:"Simple Error Handler.vi"("error in (no error)"=w18) -> ()  [unwired: 4 in, 5 out]
  }
